vi "init.vi"(8 "error in":errorcluster, 10 "TBM module configuration in":refnum<class "TBM module configuration.lvclass">, 11 "SystemLin Tag Module runtime in":refnum<class "SystemLink runtime.lvclass">) -> (0 "error out":errorcluster, 1 "data allocations":T1, 2 "execution settings":T4, 3 "SystemLin Tag Module runtime out":refnum<class "SystemLink runtime.lvclass">)   [LabVIEW 2015, in "SystemLink runtime.lvclass"]
doc: "Provides an interface for initializing a module at runtime. While this interface performs no operations, a child should provide an override which may open any necessary references or sessions, allocate necessary memory, and perform any final configuration validataion before providing the full configuration <b>execution data</b> to the calling process."
uses:
  SystemLink runtime.lvclass
  <vilib>/NI/Tag Bus Module Framework/module configuration/TBM module configuration.lvclass
  <vilib>/NI/Tag Bus Module Framework/runtime/execution settings.ctl
  <vilib>/NI/Tag Bus Module Framework/channel/data tables.ctl
  <vilib>/NI/Tag Bus/dictionary/data dictionary.lvclass
  <vilib>/NI/Tag Bus/dictionary table pair.ctl
  <vilib>/NI/Tag Bus/table/data table.ctl
  configuration/SystemLink configuration.lvclass
  configuration/SystemLink configuration.lvclass/SystemLink configuration.ctl
  SystemLink runtime.lvclass/SystemLink runtime.ctl
  configuration/SysLink Mapping.ctl
  configuration/Data Tag Type.ctl
  <vilib>/Skyline/Tag/Wrapper/Wrapper_class/NI Skyline Tag.lvclass
  <vilib>/NI/Tag Bus/tag/tag descriptor.lvclass/tag descriptor.ctl
  <vilib>/NI/Tag Bus Module Framework/channel/TBM channel.lvclass/TBM channel.ctl
  <vilib>/NI/Tag Bus/tag/read tag name.vi
  <vilib>/NI/Tag Bus Module Framework/channel/Read channel classification.vi
  <vilib>/NI/Tag Bus Module Framework/channel/TBM channel.lvclass
  <vilib>/NI/Tag Bus Module Framework/runtime/TBM module execution interface.lvclass
  <vilib>/NI/Tag Bus/tag bus.lvlib
  <vilib>/NI/Tag Bus/table/data table.lvlib
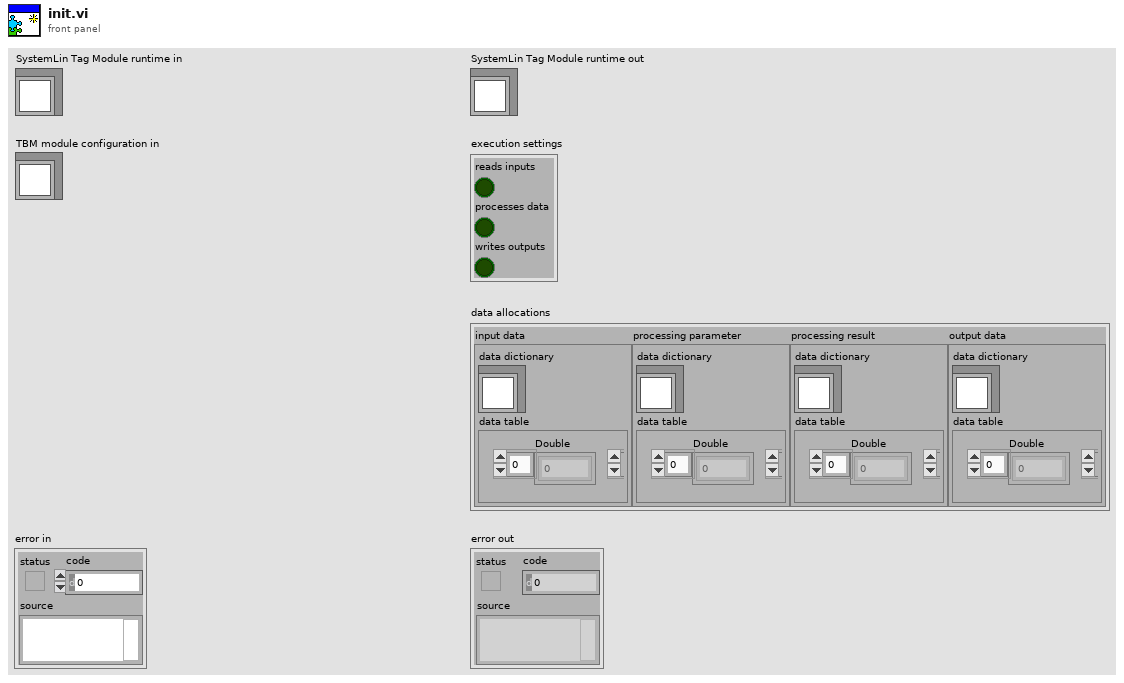
[diagram p1: front panel]
types:
  T1 = typedef "TBM channel.lvclass/data tables.ctl" = cluster{"input data":T2, "processing parameter":T2, "processing result":T2, "output data":T2}
  T2 = typedef "tag bus.lvlib/dictionary table pair.ctl" = cluster{"data dictionary":refnum<class "data dictionary.lvclass">, "data table":T3}
  T3 = typedef "tag bus.lvlib/data table.lvlib/data table.ctl" = cluster{"Double":dbl[], "Single":sgl[], "I64":i64[], "I32":i32[], "I16":i16[], "I8":i8[], "U64":u64[], "U32":u32[], "U16":u16[], "U8":u8[], "Boolean":bool[], "String":string[], "Array of Double":cluster{"DBL Array":dbl[]}[], "Array of Single":cluster{"SGL Array":sgl[]}[], "Array of I64":cluster{"I64 Array":i64[]}[], "Array of I32":cluster{"I32 Array":i32[]}[], "Array of I16":cluster{"I16 Array":i16[]}[], "Array of I8":cluster{"I8 Array":i8[]}[], "Array of U64":cluster{"U64 Array":u64[]}[], "Array of U32":cluster{"U32 Array":u32[]}[], "Array of U16":cluster{"U16 Array":u16[]}[], "Array of U8":cluster{"U8 Array":u8[]}[], "Array of Boolean":cluster{"Boolean Array":bool[]}[], "Array of String":cluster{"String Array":string[]}[]}
  T4 = typedef "TBM module execution interface.lvclass/execution settings.ctl" = cluster{"reads inputs":bool, "processes data":bool, "writes outputs":bool}
  T5 = typedef "SystemLink configuration.lvclass/SysLink Mapping.ctl" = cluster{"Data Type":T6, "Tag Reference":refnum<class "NI Skyline Tag.lvclass">, "Tag Bus Index":i32, "AMQP":bool, "Skylink Index":i32}
  T6 = typedef "SystemLink configuration.lvclass/Data Tag Type.ctl" = enum16{"Double", "Single", "I32", "I16", "I8", "U64", "U32", "U16", "U8", "Boolean", "String", "Timestamp"}
  T7 = typedef "SystemLink configuration.lvclass/Line.ctl" = cluster{"channel":refnum<class "TBM channel.lvclass">, "Data Tag Type":T6}
  T8 = typedef "SystemLink configuration.lvclass/Connection Configuration.ctl" = cluster{"Connection Type":T9, "AMQP":cluster{"Configuration ID":string}, "HTTP":cluster{"Verify Server?":bool, "Server URL":string, "CA Certificate File":string, "User Info":cluster{"Username":string, "Password":string}, "API Key":string}}
  T9 = typedef "SystemLink configuration.lvclass/Connection Type.ctl" = enum16{"AMQP", "HTTP", "API Key (SystemLink Cloud)"}
  T10 = typedef "TBM channel.lvclass/channel classification.ctl" = enum16{"input data", "output data", "processing parameter", "processing result"}
  T11 = typedef "NI Skyline Tag.lvclass/Tag Value Cluster Wrapper.ctl" = cluster{"Configuration":refnum<class "NI Skyline Configuration.lvclass">, "Tag Cluster":T12}
  T12 = typedef "NI Skyline Tag.lvlib/Tag Value Cluster.ctl" = cluster{"Path":string, "Data Type":T13, "Value":string, "Time Stamp":timestamp}
  T13 = typedef "NI Skyline Tag.lvlib/DataType.ctl" = enum32{"Double", "I32", "String", "Boolean", "U64", "Timestamp"}
  T14 = typedef "tag bus.lvlib/tag descriptor.lvclass/Data Type.ctl" = enum16{"Double", "Single", "I64", "I32", "I16", "I8", "U64", "U32", "U16", "U8", "Boolean", "String", "Array of Double", "Array of Single", "Array of I64", "Array of I32", "Array of I16", "Array of I8", "Array of U64", "Array of U32", "Array of U16", "Array of U8", "Array of Boolean", "Array of String"}
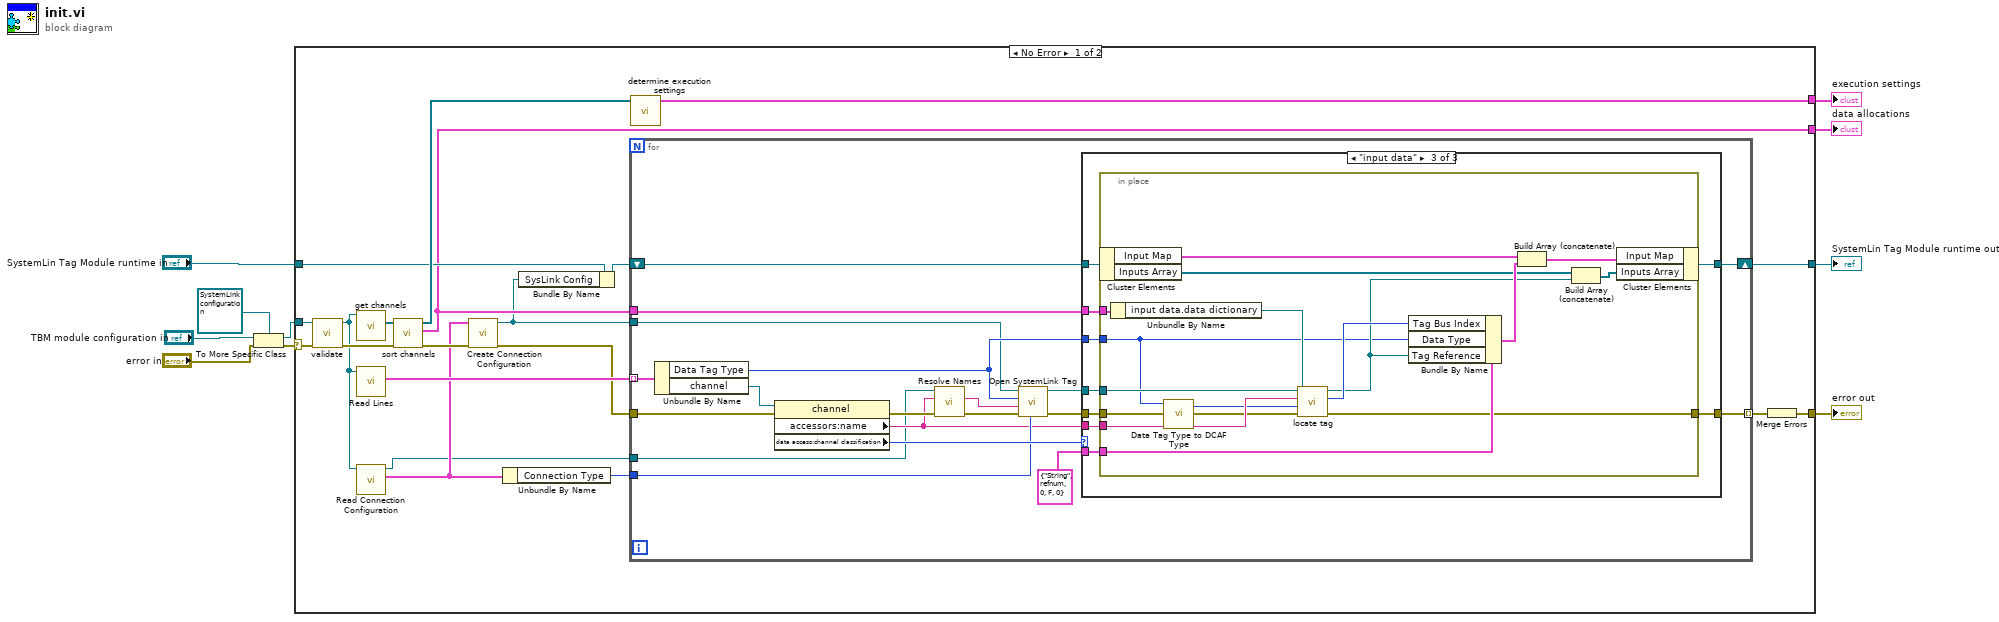
[diagram p0: block diagram]
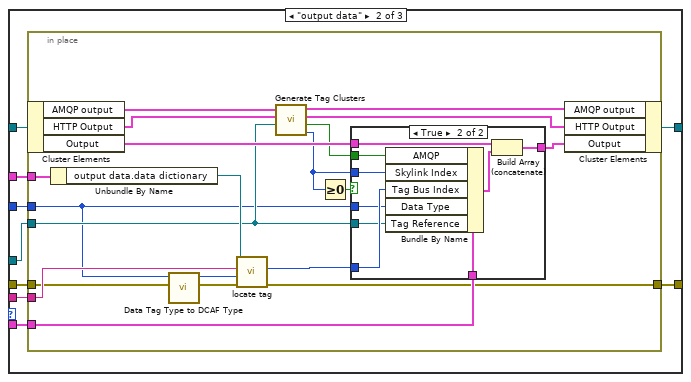
[diagram p3: hidden frame]
diagram:
  n1 = To More Specific Class(target class=refnum<class "SystemLink configuration.lvclass"> refnum ("Synchronous module configuration"), reference="TBM module configuration in", error in="error in") -> (specific class reference=w9:refnum<class "SystemLink configuration.lvclass">, error out=w10:errorcluster)
  n2 = case shown="No Error" w10 {
    selector: w10 -> [w28 w114]
    tunnel: w9 -> [w27 _]
    tunnel: "SystemLin Tag Module runtime in" -> [w24 w115]
    tunnel: [w23 w115] -> w4
    tunnel: [w19 w114] -> w3
    tunnel: [w22 _] -> w1
    tunnel: [w30 _] -> w2
    frame No Error {
      n3 = call-dynamic "validate.vi"("error in"=w28, "SystemLin Tag Module configuration in"=w27) -> ("error out"=w29:errorcluster, "SystemLin Tag Module configuration out"=w16:refnum<class "SystemLink configuration.lvclass">)  [unwired: 8 in]
      n4 = call-dynamic "get channels.vi"("SystemLin Tag Module configuration in"=w16) -> ("channels"=w26:refnum<class "TBM channel.lvclass">[])  [unwired: 9 in, 1 out]
      n5 = call "Read Lines.vi"("SystemLin Tag Module configuration in"=w16) -> ("Lines"=w18:T7[])  [unwired: 8 in, 2 out]
      n6 = call "Read Connection Configuration.vi"("SystemLink configuration in"=w16) -> ("Connection Configuration"=w15:T8, "SystemLink configuration out"=w11:refnum<class "SystemLink configuration.lvclass">)  [unwired: 8 in, 1 out]
      n7 = call <vilib>:"sort channels.vi"("error in"=w29, "channels in"=w26) -> ("error out"=w21:errorcluster, "data allocations"=w22:T1, "channels out"=w25:refnum<class "TBM channel.lvclass">[])  [unwired: 7 in]
      n8 = call "Create Connection Configuration.vi"("error in (no error)"=w21, "Connection Configuration"=w15) -> ("error out"=w17:errorcluster, "SystemLink Configuration"=w12:refnum<class "NI Skyline Configuration.lvclass">)  [unwired: 8 in]
      n9 = Unbundle By Name(w15) -> ("Connection Type"=w14:T9)
      n10 = Bundle By Name(cluster=w24, "SysLink Config"=w12) -> (w13:refnum<class "SystemLink runtime.lvclass">)
      n11 = for {
        shift-right: [w48] -> w23
        shift-left: w13 -> [w49]
        tunnel: w22 -> [w47]
        tunnel: w17 -> [w46]
        tunnel: [w45] -> w20 mode=indexing
        tunnel: w18 -> [w40] mode=indexing
        tunnel: w12 -> [w37]
        tunnel: w14 -> [w36]
        tunnel: w11 -> [w31]
        n12 = Unbundle By Name(w40) -> ("Data Tag Type"=w38:T6, "channel"=w39:refnum<class "TBM channel.lvclass">)
        n13 = property class="channel"(reference=w39, error in=w46) -> (error out=w35:errorcluster, "accessors:name"=w32:string, "data access:channel classification"=w41:T10)  [unwired: 1 out]
        n14 = call "Resolve Names.vi"("Error In"=w35, "Path In"=w32, "SystemLin Tag Module configuration"=w31) -> ("Error Out"=w34:errorcluster, "Path Out"=w33:string)  [unwired: 5 in]
        n15 = call "Open SystemLink Tag.vi"("Connection Type"=w36, "error in (no error)"=w34, "Path"=w33, "Data Tag Type"=w38, "NI Skyline Configuration in"=w37) -> ("error out"=w42:errorcluster, "NI Skyline Tag out"=w43:refnum<class "NI Skyline Tag.lvclass">)  [unwired: 5 in]
        n16 = case shown="\"input data\"" w41 {
          tunnel: w49 -> [w51 w60 w98]
          tunnel: [w51 w59 w97] -> w48
          tunnel: [w50 w58 w96] -> w45
          tunnel: w42 -> [w50 w57 w95]
          tunnel: T5 {"Data Type"=enum."String", "Tag Reference"=refnum, "Tag Bus Index"=0, "AMQP"=FALSE, "Skylink Index"=0} ("Mapping") -> [_ w56 w94]
          tunnel: w38 -> [_ w55 w93]
          tunnel: w47 -> [_ w54 w92]
          tunnel: w32 -> [_ w53 w91]
          tunnel: w43 -> [_ w52 w90]
          frame Default {
          }
          frame "output data" {
            n17 = in-place {
              in-place-border: w54 -> [w79]
              in-place-border: w53 -> [w74]
              in-place-border: w55 -> [w62]
              in-place-border: w57 -> [w73]
              in-place-border: w56 -> [w72]
              in-place-border: [w71] -> w58
              in-place-border: w52 -> [w70]
              n18 = in-place-cluster #1(w60) -> ("AMQP output"=w69:T11[], "HTTP Output"=w68:T11[], "Output"=w77:T5[])
              n19 = Unbundle By Name(w79) -> ("output data.data dictionary"=w78:refnum<class "data dictionary.lvclass">)
              n20 = call "Data Tag Type to DCAF Type.vi"("Data Tag Type"=w62) -> ("DCAF Data Type"=w61:T14)  [unwired: 10 in]
              n21 = call <vilib>:"locate tag.vi"("error in"=w73, "data type"=w61, "name"=w74, "data dictionary in"=w78) -> ("error out"=w71:errorcluster, "index"=w75:i32)  [unwired: 5 in, 1 out]
              n22 = call "Generate Tag Clusters.vi"("NI Skyline Tag in"=w70, "HTTP Output in"=w68, "AMQP output in"=w69) -> ("Index"=w63:i32, "AMQP"=w65:bool, "HTTP Output out"=w66:T11[], "AMQP output out"=w67:T11[])  [unwired: 5 in]
              n23 = Greater Or Equal To 0?(x=w63) -> (x >= 0?=w64:bool)
              n24 = case shown="True" w64 {
                tunnel: w77 -> [w80 w89]
                tunnel: [w80 w88] -> w76
                tunnel: w75 -> [_ w87]
                tunnel: w72 -> [_ w86]
                tunnel: w62 -> [_ w84]
                tunnel: w70 -> [_ w83]
                tunnel: w63 -> [_ w82]
                tunnel: w65 -> [_ w81]
                frame False {
                }
                frame True {
                  n25 = Bundle By Name(cluster=w86, "AMQP"=w81, "Skylink Index"=w82, "Tag Bus Index"=w87, "Data Type"=w84, "Tag Reference"=w83) -> (w85:T5)
                  n26 = Build Array (concatenate)(w89, w85) -> (w88:T5[])
                }
              }
              n27 = in-place-cluster #1("AMQP output"=w67, "HTTP Output"=w66, "Output"=w76) -> (w59:refnum<class "SystemLink runtime.lvclass">)
            }
          }
          frame "input data" {
            n28 = in-place {
              in-place-border: w92 -> [w113]
              in-place-border: w91 -> [w108]
              in-place-border: w93 -> [w99]
              in-place-border: w95 -> [w107]
              in-place-border: w94 -> [w106]
              in-place-border: [w105] -> w96
              in-place-border: w90 -> [w101]
              n29 = in-place-cluster #2(w98) -> ("Input Map"=w111:T5[], "Inputs Array"=w103:refnum<class "NI Skyline Tag.lvclass">[])
              n30 = Unbundle By Name(w113) -> ("input data.data dictionary"=w112:refnum<class "data dictionary.lvclass">)
              n31 = call "Data Tag Type to DCAF Type.vi"("Data Tag Type"=w99) -> ("DCAF Data Type"=w100:T14)  [unwired: 10 in]
              n32 = call <vilib>:"locate tag.vi"("error in"=w107, "data type"=w100, "name"=w108, "data dictionary in"=w112) -> ("error out"=w105:errorcluster, "index"=w109:i32)  [unwired: 5 in, 1 out]
              n33 = Bundle By Name(cluster=w106, "Tag Bus Index"=w109, "Data Type"=w99, "Tag Reference"=w101) -> (w104:T5)
              n34 = Build Array (concatenate)(w111, w104) -> (w110:T5[])
              n35 = Build Array (concatenate)(w103, w101) -> (w102:refnum<class "NI Skyline Tag.lvclass">[])
              n36 = in-place-cluster #2("Input Map"=w110, "Inputs Array"=w102) -> (w97:refnum<class "SystemLink runtime.lvclass">)
            }
          }
        }
      }
      n37 = call <vilib>:"determine execution settings.vi"("channels"=w25) -> ("execution settings"=w30:T4)  [unwired: 10 in]
      n38 = Merge Errors(w20) -> (w19:errorcluster)
    }
    frame Error {
    }
  }
  "error out" <- w3
  "SystemLin Tag Module runtime out" <- w4
  "execution settings" <- w2
  "data allocations" <- w1
